vi "Set Server State UE.vi"(10 "Server State UE":refnum<user-event>, 11 "gRPC server in":refnum<class "Servicer.lvclass">) -> (3 "gRPC server out":refnum<class "Servicer.lvclass">)   [LabVIEW 2019, in "gRPC-servicer.lvlib" / "Servicer.lvclass"]
uses:
  Servicer.lvclass
  typeDefs/Server State Data.ctl
  Servicer.lvclass/Servicer.ctl
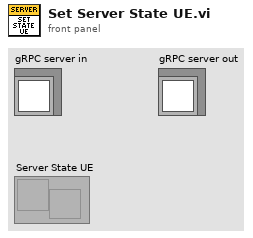
[diagram p1: front panel]
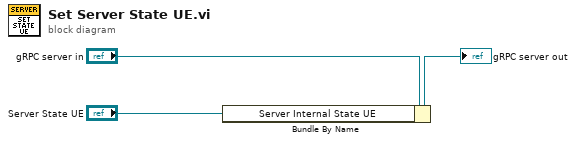
[diagram p0: block diagram]
diagram:
  n1 = Bundle By Name(cluster="gRPC server in", "Server Internal State UE"="Server State UE") -> (→"gRPC server out":refnum<class "Servicer.lvclass">)
